vi "Host_ShVariables.vi"() -> ()   [LabVIEW 2025]
panel:
  out "error IO":errorcluster
  out "Message":string
  in  "Stop Button":bool
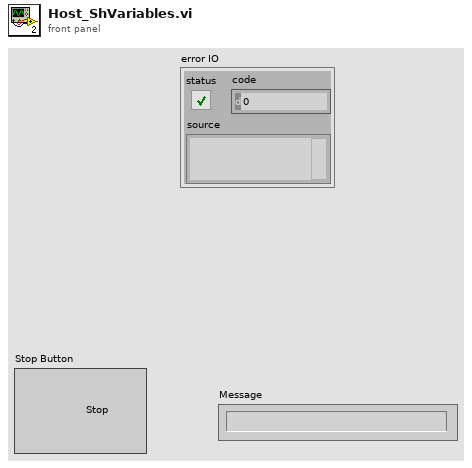
[diagram p1: front panel]
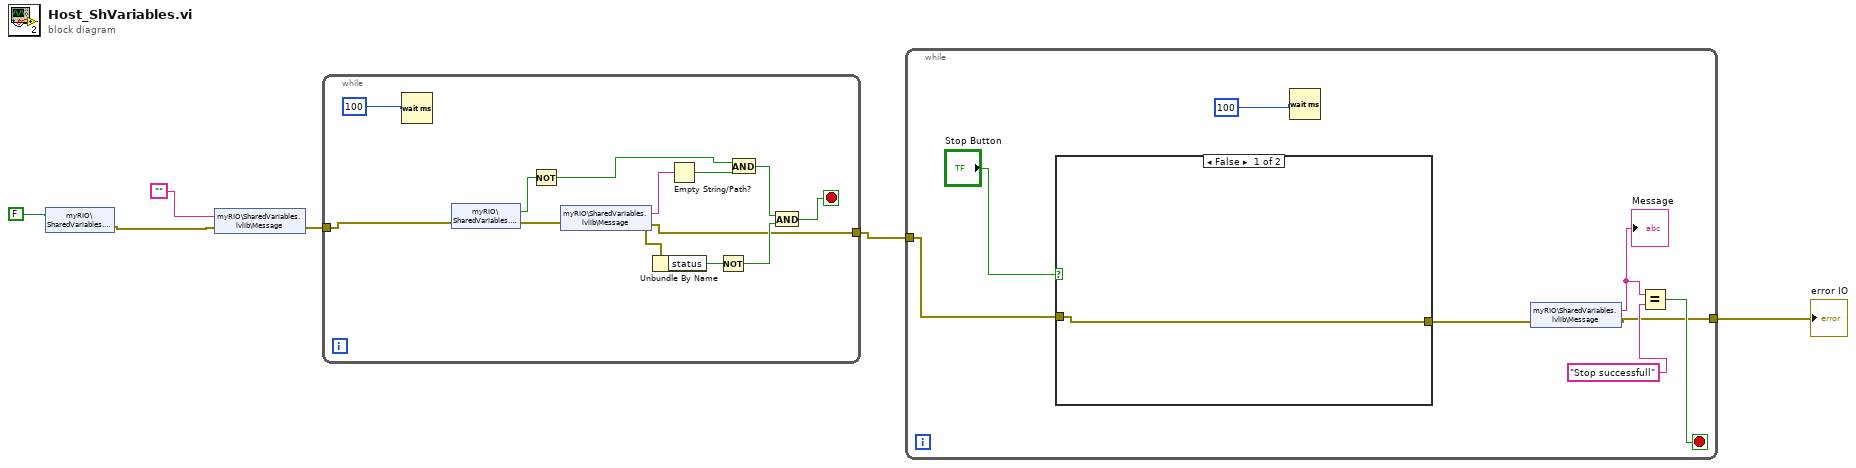
[diagram p0: block diagram]
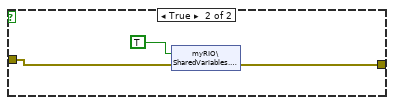
[diagram p2: hidden frame]
diagram:
  n1 = shared-variable "myRIO\\SharedVariables.lvlib\\Stop"(FALSE ("Stop")) -> (error out=w5:errorcluster)  [unwired: 1 in]
  n2 = shared-variable "myRIO\\SharedVariables.lvlib\\Message"("", error in=w5) -> (error out=w4:errorcluster)
  n3 = while {
    tunnel: w4 -> [w18]
    tunnel: [w7] -> w2
    stop <- w9 stop-if-true
    n4 = Wait (ms)(milliseconds to wait=u32 100) -> ()  [unwired: 1 out]
    n5 = shared-variable "myRIO\\SharedVariables.lvlib\\Stop"(error in=w18) -> (w16:bool, error out=w17:errorcluster)
    n6 = Not(x=w16) -> (.not. x?=w12:bool)
    n7 = shared-variable "myRIO\\SharedVariables.lvlib\\Message"(error in=w17) -> (w15:string, error out=w7:errorcluster)
    n8 = Unbundle By Name(w7) -> ("status"=w14:bool)
    n9 = Empty String/Path?(string/path=w15) -> (empty?=w13:bool)
    n10 = Not(x=w14) -> (.not. x?=w10:bool)
    n11 = And(x=w12, y=w13) -> (x .and. y?=w11:bool)
    n12 = And(x=w11, y=w10) -> (x .and. y?=w9:bool)
  }
  n13 = while {
    tunnel: w2 -> [w25]
    tunnel: [w19] -> w1
    stop <- w21 stop-if-true
    n14 = case shown="False" "Stop Button" {
      tunnel: w25 -> [w27 w30]
      tunnel: [w27 w29] -> w24
      frame False {
      }
      frame True {
        n15 = shared-variable "myRIO\\SharedVariables.lvlib\\Stop"(TRUE ("Stop"), error in=w30) -> (error out=w29:errorcluster)
      }
    }
    n16 = Wait (ms)(milliseconds to wait=u32 100) -> ()  [unwired: 1 out]
    n17 = shared-variable "myRIO\\SharedVariables.lvlib\\Message"(error in=w24) -> (w23:string, error out=w19:errorcluster)
    "Message" <- w23
    n18 = Equal?(x=w23, y="Stop successfull") -> (x = y?=w21:bool)
  }
  "error IO" <- w1
